vi "Read From File.vi"(8 "error in (no error)":errorcluster, 11 "file path":path) -> (0 "error out":errorcluster, 2 "input cfg JSON":string, 3 "input type":T1, 5 "file exists?":bool)   [LabVIEW 2022 SP3, in "input cfg file.lvlib"]
uses:
  input cfg file.lvlib
  controls/input type.ctl
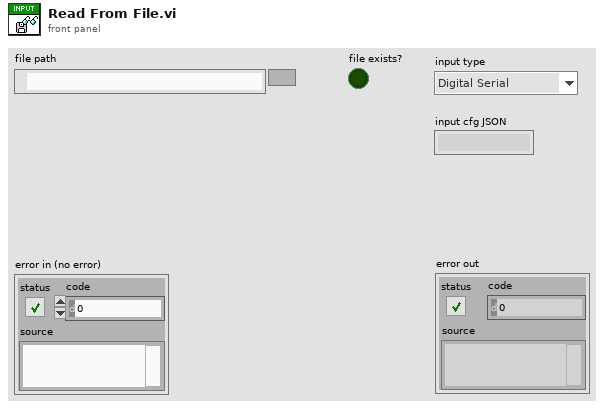
[diagram p1: front panel]
types:
  T1 = typedef "input type.ctl" = enum32{"Digital Serial", "PDM"}
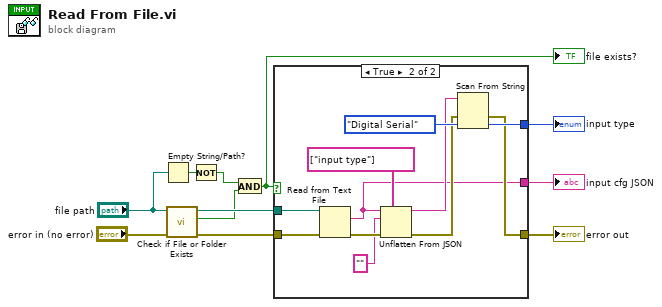
[diagram p0: block diagram]
diagram:
  n1 = Empty String/Path?(string/path="file path") -> (empty?=w2:bool)
  n2 = call <vilib>:"Check if File or Folder Exists.vi"("error in (no error)"="error in (no error)", "path"="file path") -> ("error out"=w11:errorcluster, "file or folder exists?"=w3:bool, "dup path"=w10:path)  [unwired: 7 in]
  n3 = Not(x=w2) -> (.not. x?=w1:bool)
  n4 = And(x=w1, y=w3) -> (x .and. y?=w4:bool)
  "file exists?" <- w4
  n5 = case shown="True" w4 {
    tunnel: w11 -> [w12 w22]
    tunnel: w10 -> [_ w23]
    tunnel: [w12 w14] -> w8
    tunnel: [_ w16] -> w7
    tunnel: [_ w13] -> w6
    frame False {
      # "no file found"
    }
    frame True {
      n6 = Read from Text File(file (use dialog)=w23, error in=w22) -> (text=w13:string, error out=w21:errorcluster)  [unwired: 2 in, 2 out]
      n7 = Unflatten From JSON(path=string[] ["input type"], JSON string=w13, type and defaults="", error in (no error)=w21) -> (value=w17:string, error out=w15:errorcluster)  [unwired: 3 in]
      n8 = Scan From String(input string=w17, error in=w15, default 1=input_type."Digital Serial" ("input type")) -> (error out=w14:errorcluster, output 1=w16:T1)  [unwired: 2 in, 2 out]
    }
  }
  "error out" <- w8
  "input type" <- w7
  "input cfg JSON" <- w6
